vi "Update Expression.vi"(8 "error in (no error)":errorcluster, 10 "Expression":string, 11 "Cron in":refnum<class "Cron.lvclass">) -> (0 "error out":errorcluster, 1 "valid":bool, 3 "Cron out":refnum<class "Cron.lvclass">)   [LabVIEW 2013, in "openCron.lvlib" / "Cron.lvclass"]
uses:
  Cron.lvclass
  Cron Interval -- enum.ctl
  Cron.lvclass/Cron.ctl
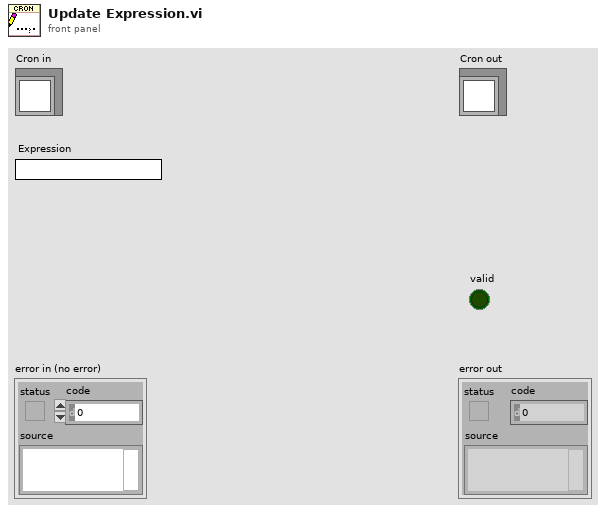
[diagram p1: front panel]
types:
  T1 = typedef "openCron.lvlib/Cron.lvclass/Cron Interval -- enum.ctl" = enum16{"Seconds", "Minutes", "Hours", "Day of Month", "Month", "Day of Week", "Year"}
  T2 = typedef "openCron.lvlib/Cron.lvclass/Cron Interval -- cluster.ctl" = cluster{"Values":i32[], "All":bool, "Any":bool}
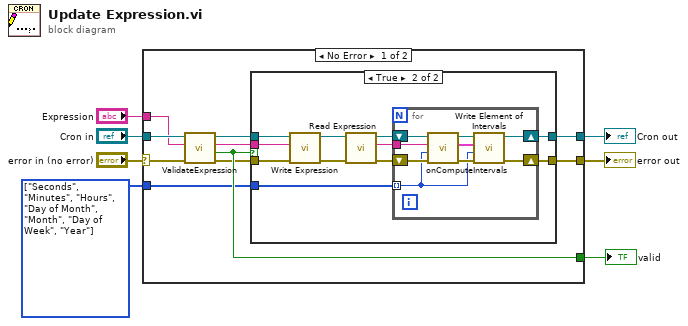
[diagram p0: block diagram]
diagram:
  w1 = T1[] [enum."Seconds", enum."Minutes", enum."Hours", enum."Day of Month", enum."Month", enum."Day of Week", enum."Year"] items=["Seconds", "Minutes", "Hours", "Day of Month", "Month", "Day of Week", "Year"]
  n1 = case shown="No Error" "error in (no error)" {
    selector: "error in (no error)" -> [w11 w40]
    tunnel: [w9 w40] -> w6
    tunnel: [w14 w41] -> w4
    tunnel: "Cron in" -> [w17 w41]
    tunnel: "Expression" -> [w15 _]
    tunnel: [w12 _] -> w2
    tunnel: w1 -> [w8 _]
    frame No Error {
      n2 = call "ValidateExpression.vi"("error in (no error)"=w11, "Expression"=w15, "Cron in"=w17) -> ("error out"=w10:errorcluster, "valid?"=w12:bool, "Expression dup"=w13:string, "Cron out"=w16:refnum<class "Cron.lvclass">)  [unwired: 5 in]
      n3 = case shown="True" w12 {
        tunnel: w16 -> [w19 w30]
        tunnel: [w19 w22] -> w14
        tunnel: w13 -> [_ w29]
        tunnel: w10 -> [w18 w28]
        tunnel: [w18 w21] -> w9
        tunnel: w8 -> [_ w20]
        frame False {
        }
        frame True {
          n4 = call "Write Expression.vi"("error in (no error)"=w28, "Expression"=w29, "Cron in"=w30) -> ("error out"=w25:errorcluster, "Cron out"=w27:refnum<class "Cron.lvclass">)  [unwired: 7 in]
          n5 = call "Read Expression.vi"("error in (no error)"=w25, "Cron in"=w27) -> ("error out"=w24:errorcluster, "Expression"=w23:string, "Cron out"=w26:refnum<class "Cron.lvclass">)  [unwired: 7 in]
          n6 = for {
            tunnel: w23 -> [w37]
            shift-right: [w35] -> w22
            shift-left: w26 -> [w39]
            shift-right: [w33] -> w21
            shift-left: w24 -> [w38]
            tunnel: w20 -> [w31] mode=indexing
            n7 = call-dynamic "onComputeIntervals.vi"("error in (no error)"=w38, "Cron Interval"=w31, "Expression"=w37, "Cron in"=w39) -> ("error out"=w34:errorcluster, "Interval Parameters"=w32:T2, "Cron out"=w36:refnum<class "Cron.lvclass">)  [unwired: 5 in]
            n8 = call "Write Element of Intervals.vi"("error in (no error)"=w34, "Interval"=w31, "Parameters"=w32, "Cron in"=w36) -> ("error out"=w33:errorcluster, "Cron out"=w35:refnum<class "Cron.lvclass">)  [unwired: 6 in]
          }
        }
      }
    }
    frame Error {
    }
  }
  "error out" <- w6
  "Cron out" <- w4
  "valid" <- w2
